vi "test_Move to 360 and 0 with Return Speed.vi"(8 "error in (no error)":errorcluster, 11 "TestCase in":refnum<class "EM1000 Turn Table.lvclass">) -> (0 "error out":errorcluster, 3 "TestCase out":refnum<class "EM1000 Turn Table.lvclass">)   [LabVIEW 2020, in "EM1000 Turn Table.lvclass"]
uses:
  EM1000 Turn Table.lvclass
  EM1000 Turn Table.lvclass/EM1000 Turn Table.ctl
  <vilib>/addons/_JKI Toolkits/VI Tester/TestCase.llb/TestCase.lvclass
  AUDIX EM1000.lvclass
  C:/Program Files (x86)/National Instruments/LabVIEW 2020/vi.lib/addons/_JKI Toolkits/VI Tester/TestCase.llb/TestCase.lvclass
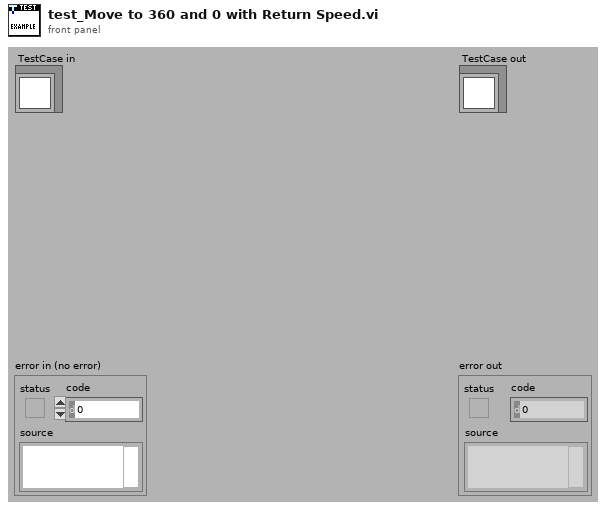
[diagram p1: front panel]
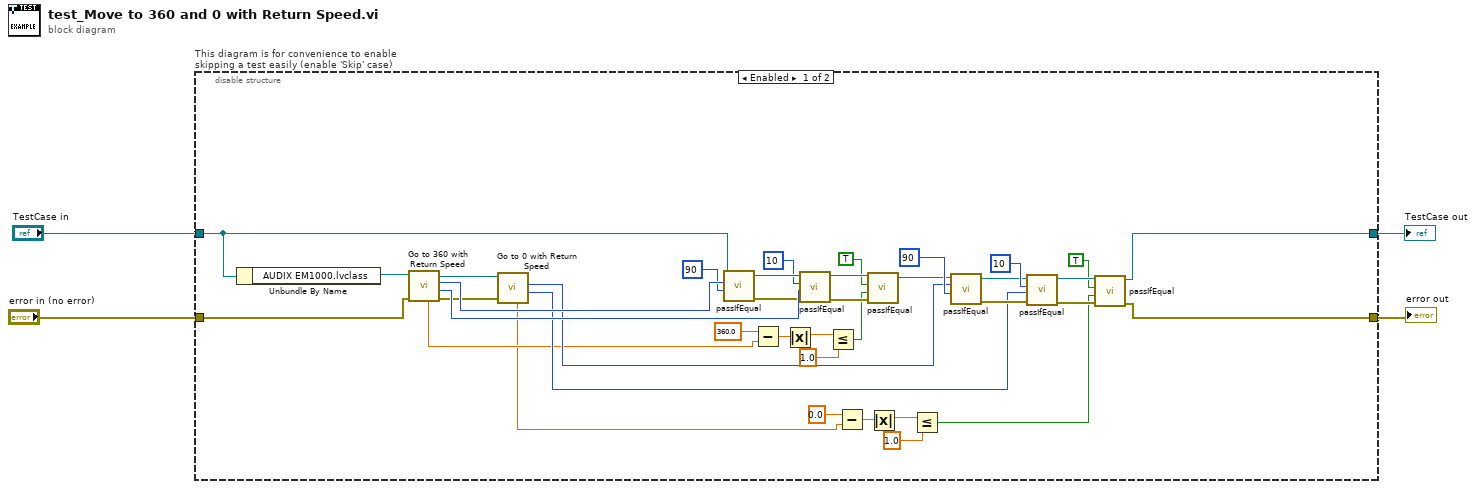
[diagram p0: block diagram]
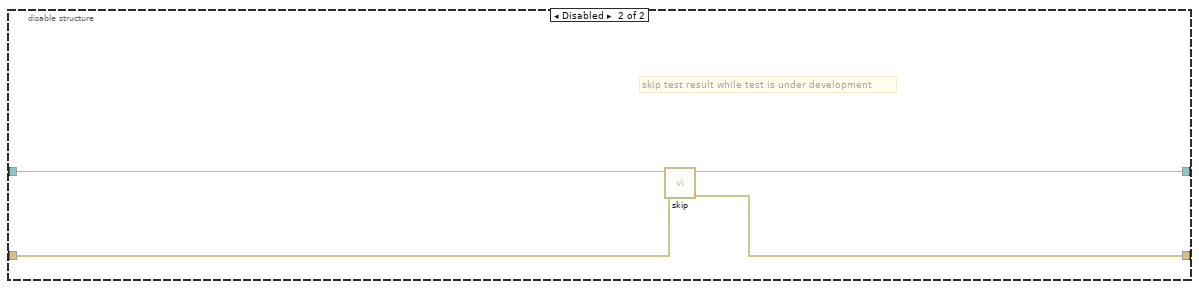
[diagram p2: hidden frame]
diagram:
  n1 = disable-structure "This diagram is for convenience to enable skipping a test easily (enable 'Skip' case)" shown="Enabled" {
    disable-tunnel: "TestCase in" -> [w33 w46]
    disable-tunnel: [w20 w44] -> w1
    disable-tunnel: [w19 w45] -> w3
    disable-tunnel: "error in (no error)" -> [w32 w43]
    frame Enabled {
      n2 = Unbundle By Name(w33) -> ("AUDIX EM1000.lvclass"=w42:refnum<class "AUDIX EM1000.lvclass">)
      n3 = call "Go to 360 with Return Speed.vi"("error in (no error)"=w32, "AUDIX EM1000 in"=w42) -> ("error out"=w30:errorcluster, "Final Speed"=w38:i32, "Return Speed"=w41:i32, "AUDIX EM1000 out"=w31:refnum<class "AUDIX EM1000.lvclass">, "TT Angle"=w17:dbl)  [unwired: 5 in]
      n4 = call "Go to 0 with Return Speed.vi"("error in (no error)"=w30, "AUDIX EM1000 in"=w31) -> ("Final Speed"=w21:i32, "Return Speed"=w22:i32, "TT Angle"=w7:dbl)  [unwired: 5 in, 2 out]
      n5 = call-dynamic "passIfEqual.vi"("y"=90, "x"=w41, "TestCase in"=w33) -> ("error out"=w35:errorcluster, "TestCase out"=w39:refnum<class "EM1000 Turn Table.lvclass">)  [unwired: 7 in]
      n6 = Subtract(x=360.0, y=w17) -> (x-y=w16:dbl)
      n7 = Absolute Value(x=w16) -> (abs(x)=w15:dbl)
      n8 = call-dynamic "passIfEqual.vi"("error in (no error)"=w35, "y"=w38, "x"=10, "TestCase in"=w39) -> ("error out"=w34:errorcluster, "TestCase out"=w36:refnum<class "EM1000 Turn Table.lvclass">)  [unwired: 6 in]
      n9 = Less Or Equal?(x=w15, y=1.0) -> (x <= y?=w13:bool)
      n10 = Subtract(x=0.0, y=w7) -> (x-y=w9:dbl)
      n11 = call-dynamic "passIfEqual.vi"("error in (no error)"=w34, "y"=w13, "x"=TRUE, "TestCase in"=w36) -> ("TestCase out"=w23:refnum<class "EM1000 Turn Table.lvclass">)  [unwired: 6 in, 1 out]
      n12 = Absolute Value(x=w9) -> (abs(x)=w10:dbl)
      n13 = Less Or Equal?(x=w10, y=1.0) -> (x <= y?=w6:bool)
      n14 = call-dynamic "passIfEqual.vi"("y"=90, "x"=w22, "TestCase in"=w23) -> ("error out"=w28:errorcluster, "TestCase out"=w25:refnum<class "EM1000 Turn Table.lvclass">)  [unwired: 7 in]
      n15 = call-dynamic "passIfEqual.vi"("error in (no error)"=w28, "y"=w21, "x"=10, "TestCase in"=w25) -> ("error out"=w29:errorcluster, "TestCase out"=w27:refnum<class "EM1000 Turn Table.lvclass">)  [unwired: 6 in]
      n16 = call-dynamic "passIfEqual.vi"("error in (no error)"=w29, "y"=w6, "x"=TRUE, "TestCase in"=w27) -> ("error out"=w19:errorcluster, "TestCase out"=w20:refnum<class "EM1000 Turn Table.lvclass">)  [unwired: 6 in]
    }
    frame Disabled {
      # "skip test result while test is under development"
      n17 = call <vilib>:"skip.vi"("error in (no error)"=w43, "TestCase in"=w46) -> ("error out"=w45:errorcluster, "TestCase out"=w44:refnum<class "EM1000 Turn Table.lvclass">)  [unwired: 8 in]
    }
  }
  "error out" <- w3
  "TestCase out" <- w1
